vi "Login - Copy.vi"(8 "error in (no error)":errorcluster) -> (0 "error out":errorcluster, 3 "Access":T1)   [LabVIEW 2021]
uses:
  Control/Access.ctl
  Control/Ini.ctl
  controls/Password check.ctl
panel:
  in  "Back Button":bool
  out "PASSWORD 2":string
  out "LOG ID 2":string
  in  "Tab Control":enum32{"Page 1", "Page 2", "Page 3"}(tab)
  in  "Operator":bool
  in  "engineer":bool
  in  "Admin":bool
  in  "LOG ID":string
  in  "OK":bool caption="OK2"
  in  "PASSWORD":string
  in  "LOG ID":string
  in  "OK":bool caption="OK2"
  # "PLEASE SELECT THE USER TYPE"
  # "Enter opertor Name and ID\n and press OK"
  # "Enter opertor Name and ID\n and press OK"
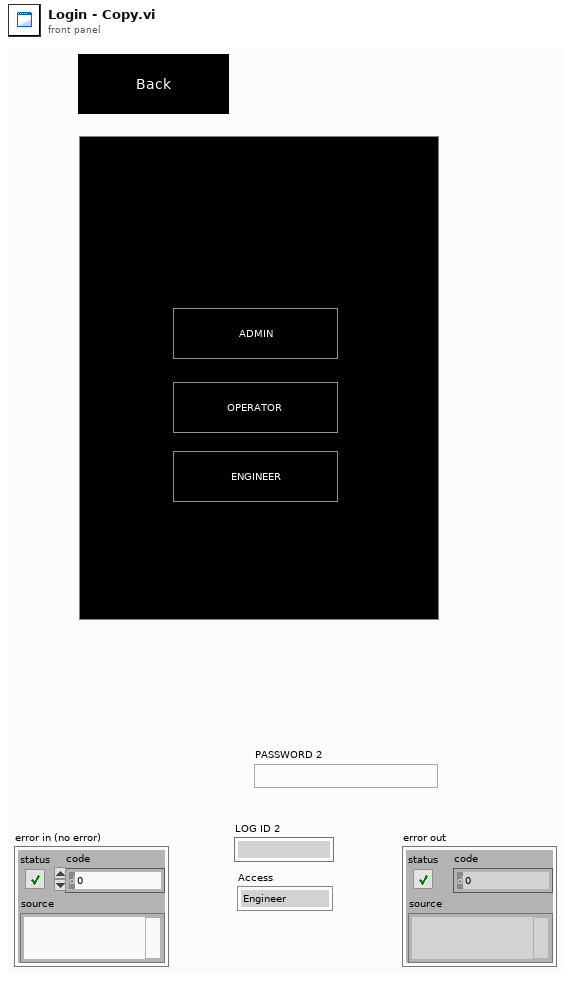
[diagram p1: front panel]
types:
  T1 = typedef "Access.ctl" = enum16{"Engineer", "Operator", "Admin"}
  T2 = typedef "Ini.ctl" = enum16{"Write", "Read"}
  T3 = typedef "Password check.ctl" = enum16{"Enter Password", "Password verification", "Exit"}
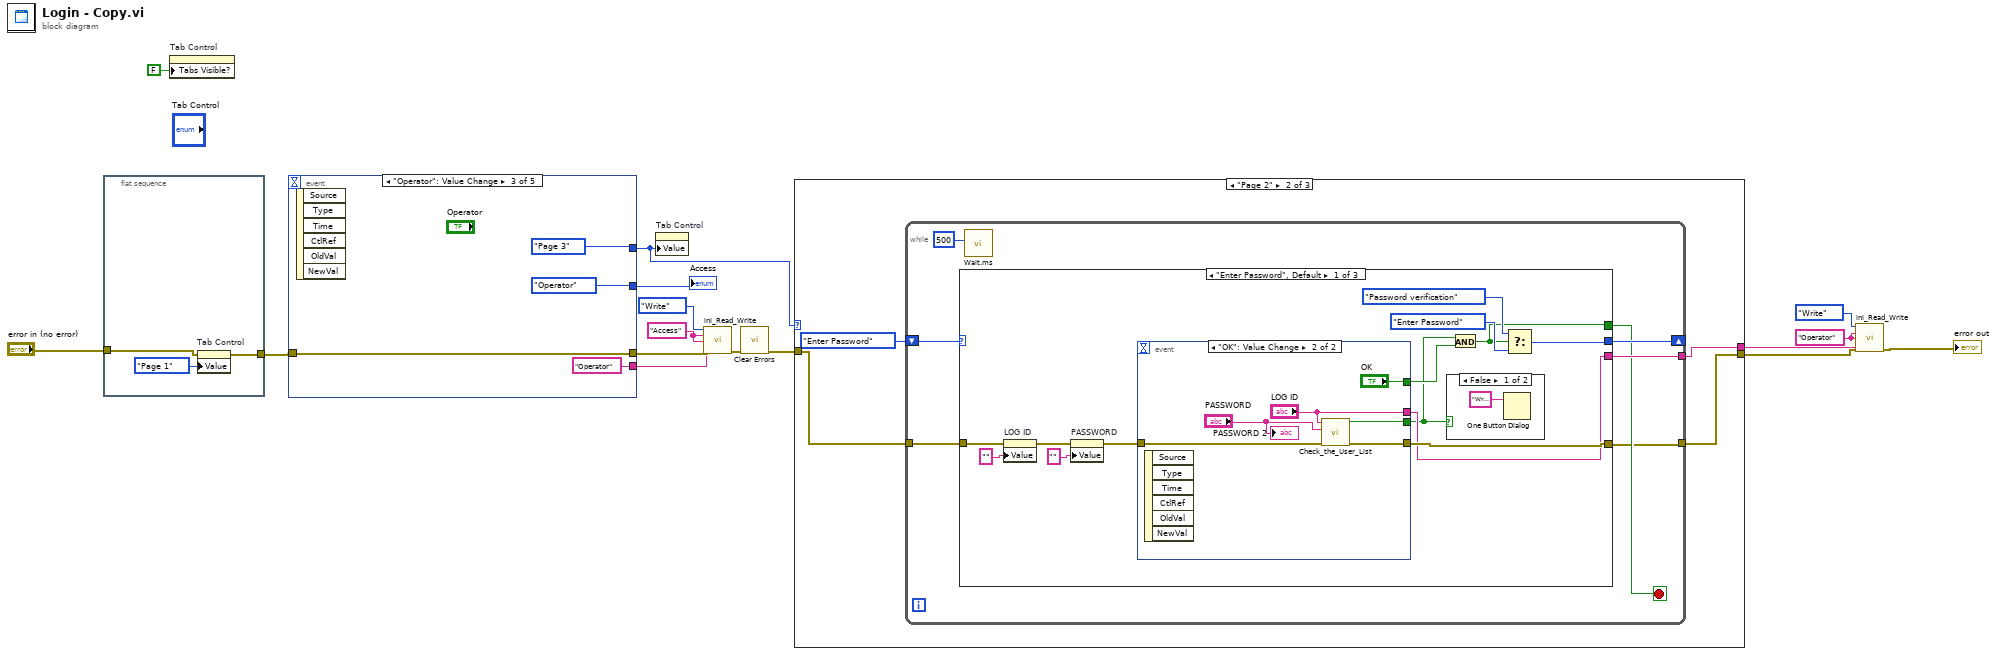
[diagram p0: block diagram]
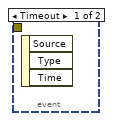
[diagram p3: hidden frame]
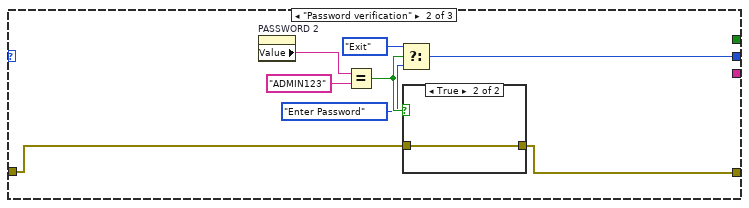
[diagram p5: hidden frame]
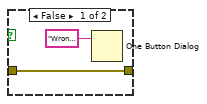
[diagram p6: hidden frame]
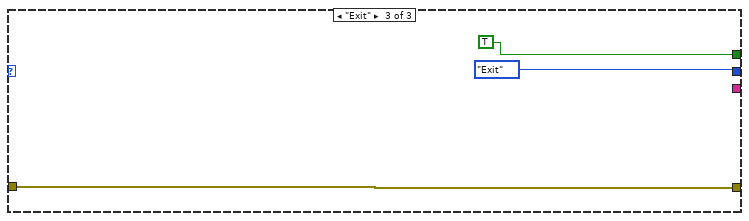
[diagram p7: hidden frame]
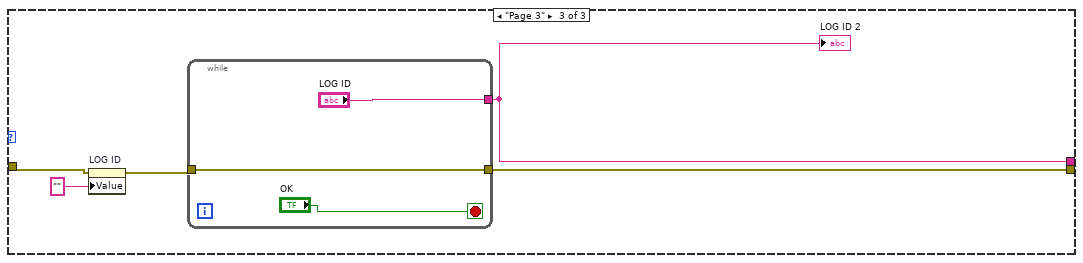
[diagram p8: hidden frame]
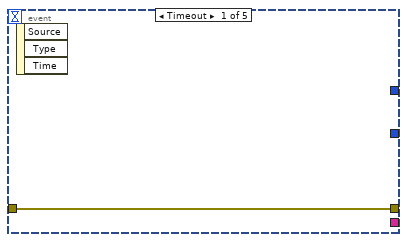
[diagram p9: hidden frame]
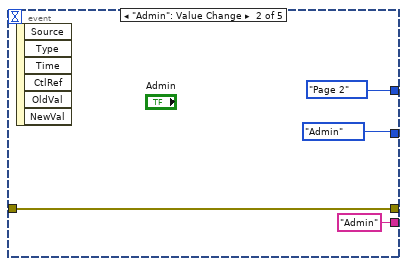
[diagram p10: hidden frame]
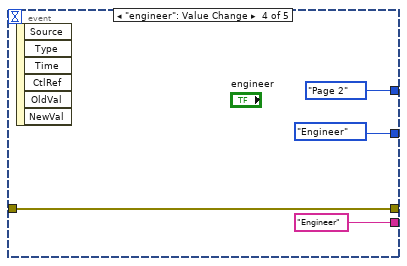
[diagram p11: hidden frame]
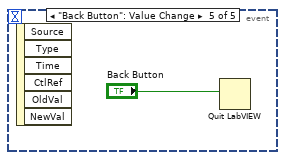
[diagram p12: hidden frame]
diagram:
  w6 = "Operator" ("Write Section")
  w10 = "Access" ("Write")
  n1 = flat-sequence {
    tunnel: [w19] -> w1
    tunnel: "error in (no error)" -> [w18]
    frame #0 {
      n2 = property on="Tab Control" class="TabCtl (strict)"(error in=w18, "Value"=enum32{"Page 1", "Page 2", "Page 3"}."Page 1" ("Tab Control")) -> (error out=w19:errorcluster)  [unwired: 1 in, 1 out]
    }
  }
  n3 = property on="Tab Control" class="TabCtl (strict)"("Tabs Visible?"=FALSE) -> ()  [unwired: 2 in, 2 out]
  n4 = event shown="[2] \"Operator\": Value Change" {
    selector: _ -> [_ _ _ _ _]
    dyn-events: _ -> [_ _ _ _ _]
    timeout: _ -> [_ _ _ _ _]
    tunnel: [_ enum16{"Engineer", "Operator", "Admin"}."Admin" enum16{"Engineer", "Operator", "Admin"}."Operator" enum16{"Engineer", "Operator", "Admin"}."Engineer" _] -> w16
    tunnel: w1 -> [w20 w23 w27 w31 _]
    tunnel: [w20 w23 w27 w31 _] -> w13
    tunnel: [_ "Admin" ("Write") "Operator" ("Write") "Engineer" ("Write") _] -> w11
    tunnel: [_ enum32{"Page 1", "Page 2", "Page 3"}."Page 2" ("Tab Control") enum32{"Page 1", "Page 2", "Page 3"}."Page 3" ("Tab Control") enum32{"Page 1", "Page 2", "Page 3"}."Page 2" ("Tab Control") _] -> w4
    event Timeout {
      n5 = event-data() -> ()  [unwired: 1 in, 3 out]
    }
    event "Admin": Value Change {
      n6 = event-data() -> ()  [unwired: 1 in, 6 out]
    }
    event "Operator": Value Change {
      n7 = event-data() -> ()  [unwired: 1 in, 6 out]
    }
    event "engineer": Value Change {
      n8 = event-data() -> ()  [unwired: 1 in, 6 out]
    }
    event "Back Button": Value Change {
      n9 = event-data() -> ()  [unwired: 1 in, 6 out]
      n10 = Quit LabVIEW(quit? (T)="Back Button") -> ()
    }
  }
  "Access" <- w16
  n11 = property on="Tab Control" class="TabCtl (strict)"("Value"=w4) -> ()  [unwired: 2 in, 2 out]
  n12 = call "ini_Read_Write.vi"(0:Ini."Write", "Write Section"=w10, "Write key"=w10, "Write"=w11, "error in (no error) 2"=w13) -> ("error in (no error) 3"=w3:errorcluster)  [unwired: 9 in, 1 out]
  n13 = call <vilib>:"Clear Errors.vi"("error in (no error)"=w3) -> ("error out"=w2:errorcluster)  [unwired: 5 in, 1 out]
  n14 = case shown="\"Page 2\"" w4 {
    tunnel: w2 -> [w34 w37 w81]
    tunnel: [w34 w35 w84] -> w9
    tunnel: [_ w38 w83] -> w5
    frame "Page 1", Default {
    }
    frame "Page 2" {
      n15 = while {
        tunnel: [w45] -> w38
        tunnel: w37 -> [w41]
        shift-right: [w43] -> _
        shift-left: Password_check."Enter Password" ("Enum") -> [w44]
        tunnel: [w40] -> w35
        stop <- w42 stop-if-true
        n16 = case shown="\"Enter Password\", Default" w44 {
          tunnel: [w54 _ _] -> w45
          tunnel: [w56 w68 Password_check."Exit" ("f")] -> w43
          tunnel: [w51 _ TRUE] -> w42
          tunnel: w41 -> [w47 w67 w77]
          tunnel: [w55 w66 w77] -> w40
          frame "Enter Password", Default {
            n17 = property on="LOG ID" class="Str"(error in=w47, "Value"="" ("LOG ID")) -> (error out=w50:errorcluster)  [unwired: 1 in, 1 out]
            n18 = property on="PASSWORD" class="Str"(error in=w50, "Value"="" ("PASSWORD")) -> (error out=w46:errorcluster)  [unwired: 1 in, 1 out]
            n19 = event shown="[1] \"OK\": Value Change" {
              selector: _ -> [_ _]
              dyn-events: _ -> [_ _]
              timeout: _ -> [_ _]
              tunnel: w46 -> [_ w64]
              tunnel: [_ w63] -> w55
              tunnel: [_ w62] -> w52
              tunnel: [_ "LOG ID"] -> w54
              tunnel: [_ "OK"] -> w53
              event Timeout {
                n20 = event-data() -> ()  [unwired: 1 in, 3 out]
              }
              event "OK": Value Change {
                n21 = event-data() -> ()  [unwired: 1 in, 6 out]
                n22 = call "Check_the_User_List.vi"("error in (no error)"=w64, "Password"="PASSWORD", "Name"="LOG ID") -> ("error out"=w63:errorcluster, "Result"=w62:bool)  [unwired: 7 in]
                "PASSWORD 2" <- "PASSWORD"
              }
            }
            n23 = case shown="False" w52 {
              frame False {
                n24 = One Button Dialog(message="Wrong Password or User ID ") -> ()  [unwired: 1 in, 1 out]
              }
              frame True {
              }
            }
            n25 = And(x=w52, y=w53) -> (x .and. y?=w51:bool)
            n26 = Select(t=Password_check."Password verification" ("Enum"), s=w51, f=Password_check."Enter Password") -> (s? t:f=w56:T3)
          }
          frame "Password verification" {
            n27 = property on="PASSWORD 2" class="Str"() -> ("Value"=w73:string)  [unwired: 2 in, 2 out]
            n28 = Equal?(x=w73, y="ADMIN123") -> (x = y?=w71:bool)
            n29 = Select(t=Password_check."Exit" ("Enum"), s=w71, f=Password_check."Enter Password") -> (s? t:f=w68:T3)
            n30 = case shown="True" w71 {
              tunnel: w67 -> [w74 w76]
              tunnel: [w74 w76] -> w66
              frame False {
                n31 = One Button Dialog(message="Wrong Password") -> ()  [unwired: 1 in, 1 out]
              }
              frame True {
              }
            }
          }
          frame "Exit" {
          }
        }
        n32 = call "Wait.ms.vi"("milliseconds to wait"=u32 500) -> ()  [unwired: 10 in, 1 out]
      }
    }
    frame "Page 3" {
      n33 = property on="LOG ID" class="Str"(error in=w81, "Value"="" ("LOG ID")) -> (error out=w80:errorcluster)  [unwired: 1 in, 1 out]
      n34 = while {
        tunnel: ["LOG ID"] -> w83
        tunnel: w80 -> [w87]
        tunnel: [w87] -> w84
        stop <- "OK" stop-if-true
      }
      "LOG ID 2" <- w83
    }
  }
  n35 = call "ini_Read_Write.vi"(0:Ini."Write", "Write Section"=w6, "Write key"=w6, "Write"=w5, "error in (no error) 2"=w9) -> ("error in (no error) 3"=→"error out":errorcluster)  [unwired: 9 in, 1 out]
